vi "init.vi"(8 "error in":errorcluster, 10 "TBM module configuration in":refnum<class "TBM module configuration.lvclass">, 11 "Daqmx Module runtime in":refnum<class "Daqmx Module runtime.lvclass">) -> (0 "error out":errorcluster, 1 "data allocations":T1, 2 "execution settings":T4, 3 "Daqmx Module runtime out":refnum<class "Daqmx Module runtime.lvclass">)   [LabVIEW 2015, in "DAQmx Module Runtime.lvclass"]
doc: "Provides an interface for initializing a module at runtime. While this interface performs no operations, a child should provide an override which may open any necessary references or sessions, allocate necessary memory, and perform any final configuration validataion before providing the full configuration <b>execution data</b> to the calling process."
uses:
  Daqmx Module runtime.lvclass
  <vilib>/NI/Tag Bus Module Framework/module configuration/TBM module configuration.lvclass
  <vilib>/NI/Tag Bus Module Framework/runtime/execution settings.ctl
  <vilib>/NI/Tag Bus Module Framework/channel/data tables.ctl
  <vilib>/NI/Tag Bus/dictionary/data dictionary.lvclass
  <vilib>/NI/Tag Bus/dictionary table pair.ctl
  <vilib>/NI/Tag Bus/table/data table.ctl
  configuration/Daqmx Module configuration.lvclass
  Channel Indeces.ctl
  configuration/Daqmx Module configuration.lvclass/Daqmx Module configuration.ctl
  <vilib>/NI/Tag Bus/tag/tag descriptor.lvclass/tag descriptor.ctl
  Daqmx Module runtime.lvclass/Daqmx Module runtime.ctl
  configuration/Read Data Rate.vi
  <vilib>/NI/Tag Bus/tag/read tag name.vi
  <vilib>/NI/Tag Bus/tag/read data type.vi
  <vilib>/NI/Tag Bus/dictionary/locate tag.vi
  <vilib>/DAQmx/create/channels.llb/DAQmx Create Channel (AI-Voltage-Basic).vi
  <vilib>/DAQmx/create/channels.llb/DAQmx Create Channel (AI-Strain-Strain Gage).vi
  <vilib>/DAQmx/create/channels.llb/DAQmx Create Channel (AI-Temperature-Thermocouple).vi
  <vilib>/DAQmx/create/channels.llb/DAQmx Create Channel (AI-Current-Basic).vi
  <vilib>/DAQmx/create/channels.llb/DAQmx Create Channel (AI-Temperature-RTD).vi
  <vilib>/DAQmx/create/channels.llb/DAQmx Create Channel (AO-Current-Basic).vi
  <vilib>/DAQmx/create/channels.llb/DAQmx Create Channel (AO-Voltage-Basic).vi
  <vilib>/DAQmx/create/channels.llb/DAQmx Create Channel (DO-Digital Output).vi
  <vilib>/DAQmx/create/channels.llb/DAQmx Create Channel (CO-Pulse Generation-Frequency).vi
  <vilib>/DAQmx/create/channels.llb/DAQmx Create Channel (DI-Digital Input).vi
  <vilib>/NI/Tag Bus Module Framework/channel/TBM channel.lvclass
  <vilib>/NI/Tag Bus Module Framework/runtime/TBM module execution interface.lvclass
  <resource>/objmgr/daqmx.rc
  <vilib>/NI/Tag Bus/tag bus.lvlib
  <vilib>/NI/Tag Bus/table/data table.lvlib
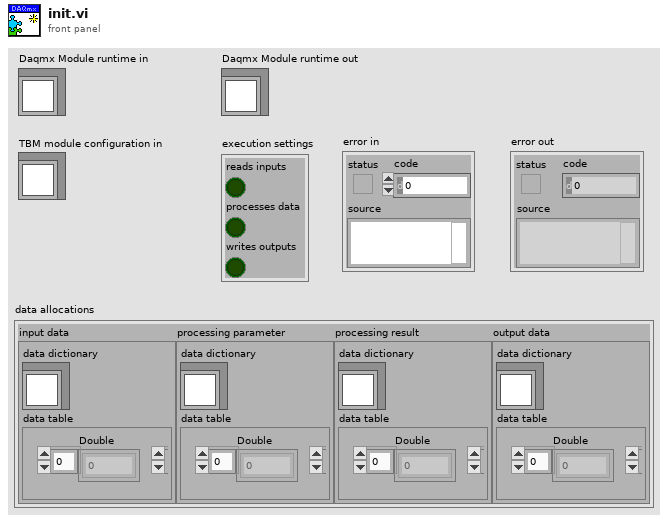
[diagram p1: front panel]
types:
  T1 = typedef "TBM channel.lvclass/data tables.ctl" = cluster{"input data":T2, "processing parameter":T2, "processing result":T2, "output data":T2}
  T2 = typedef "tag bus.lvlib/dictionary table pair.ctl" = cluster{"data dictionary":refnum<class "data dictionary.lvclass">, "data table":T3}
  T3 = typedef "tag bus.lvlib/data table.lvlib/data table.ctl" = cluster{"Double":dbl[], "Single":sgl[], "I64":i64[], "I32":i32[], "I16":i16[], "I8":i8[], "U64":u64[], "U32":u32[], "U16":u16[], "U8":u8[], "Boolean":bool[], "String":string[], "Array of Double":cluster{"DBL Array":dbl[]}[], "Array of Single":cluster{"SGL Array":sgl[]}[], "Array of I64":cluster{"I64 Array":i64[]}[], "Array of I32":cluster{"I32 Array":i32[]}[], "Array of I16":cluster{"I16 Array":i16[]}[], "Array of I8":cluster{"I8 Array":i8[]}[], "Array of U64":cluster{"U64 Array":u64[]}[], "Array of U32":cluster{"U32 Array":u32[]}[], "Array of U16":cluster{"U16 Array":u16[]}[], "Array of U8":cluster{"U8 Array":u8[]}[], "Array of Boolean":cluster{"Boolean Array":bool[]}[], "Array of String":cluster{"String Array":string[]}[]}
  T4 = typedef "TBM module execution interface.lvclass/execution settings.ctl" = cluster{"reads inputs":bool, "processes data":bool, "writes outputs":bool}
  T5 = typedef "DAQmx Module Runtime.lvclass/Channel Indeces.ctl" = cluster{"AI Index":i32[], "AO Index":i32[], "DI Index":i32[], "DO Index":i32[], "PWM Freq Index":i32[], "PWM DC Index":i32[]}
  T6 = typedef "DAQmx Module Configuration.lvclass/Line.ctl" = cluster{"Channel Array":refnum<class "TBM channel.lvclass">[], "Physical Channel":string, "Measurement Type":T7, "Parameters":T8}
  T7 = typedef "DAQmx Module Configuration.lvclass/Measurement Type.ctl" = enum16{"Digital Input", "Digital Output", "Voltage Input", "Voltage Output", "Current Input", "Current Output", "RTD", "Thermocouple", "Strain", "PWM"}
  T8 = typedef "DAQmx Module Configuration.lvclass/Parameters.ctl" = cluster{"Digital Config":cluster{"Invert Lines?":bool}, "Voltage Config":cluster{"Maximum Value (V)":dbl, "Minimum Value (V)":dbl, "in terminal configuration (V)":i32, "out terminal configuration (V)":i32}, "Current Config":cluster{"Maximum Value (A)":dbl, "Minimum Value (A)":dbl, "shunt resistor location":i32, "input terminal configuration (C)":i32, "external shunt resistor value":dbl}, "RTD Config":cluster{"Maximum Value (°C)":dbl, "Minimum Value (°C)":dbl, "resistance configuration":i32, "r0":dbl, "current excitation value":dbl, "rtd type":i32, "current excitation source":i32}, "Thermocouple Config":cluster{"Minimum Value (C)":dbl, "Maximum Value (C)":dbl, "thermocouple type":i32, "cjc source":i32, "cjc value":dbl}, "Strain Config":cluster{"Maximum Value":dbl, "Minimum Value":dbl, "bridge information":cluster{"strain configuration":i32, "lead wire resistance":dbl, "initial bridge voltage":dbl, "voltage excitation source":i32, "voltage excitation value":dbl}, "strain gage information":cluster{"gage factor":dbl, "nominal gage resistance":dbl, "poisson ratio":dbl}}, "PWM Config":cluster{"Idle State":bool}}
  T9 = typedef "DAQmx Module Runtime.lvclass/DAQ Tasks.ctl" = cluster{"AI Task":refnum<k21>, "AO Task":refnum<k21>, "DI Task":refnum<k21>, "DO Task":refnum<k21>, "PWM Task":refnum<k21>}
  T10 = cluster{"strain configuration":i32, "lead wire resistance":dbl, "initial bridge voltage":dbl, "voltage excitation source":i32, "voltage excitation value":dbl}
  T11 = cluster{"gage factor":dbl, "nominal gage resistance":dbl, "poisson ratio":dbl}
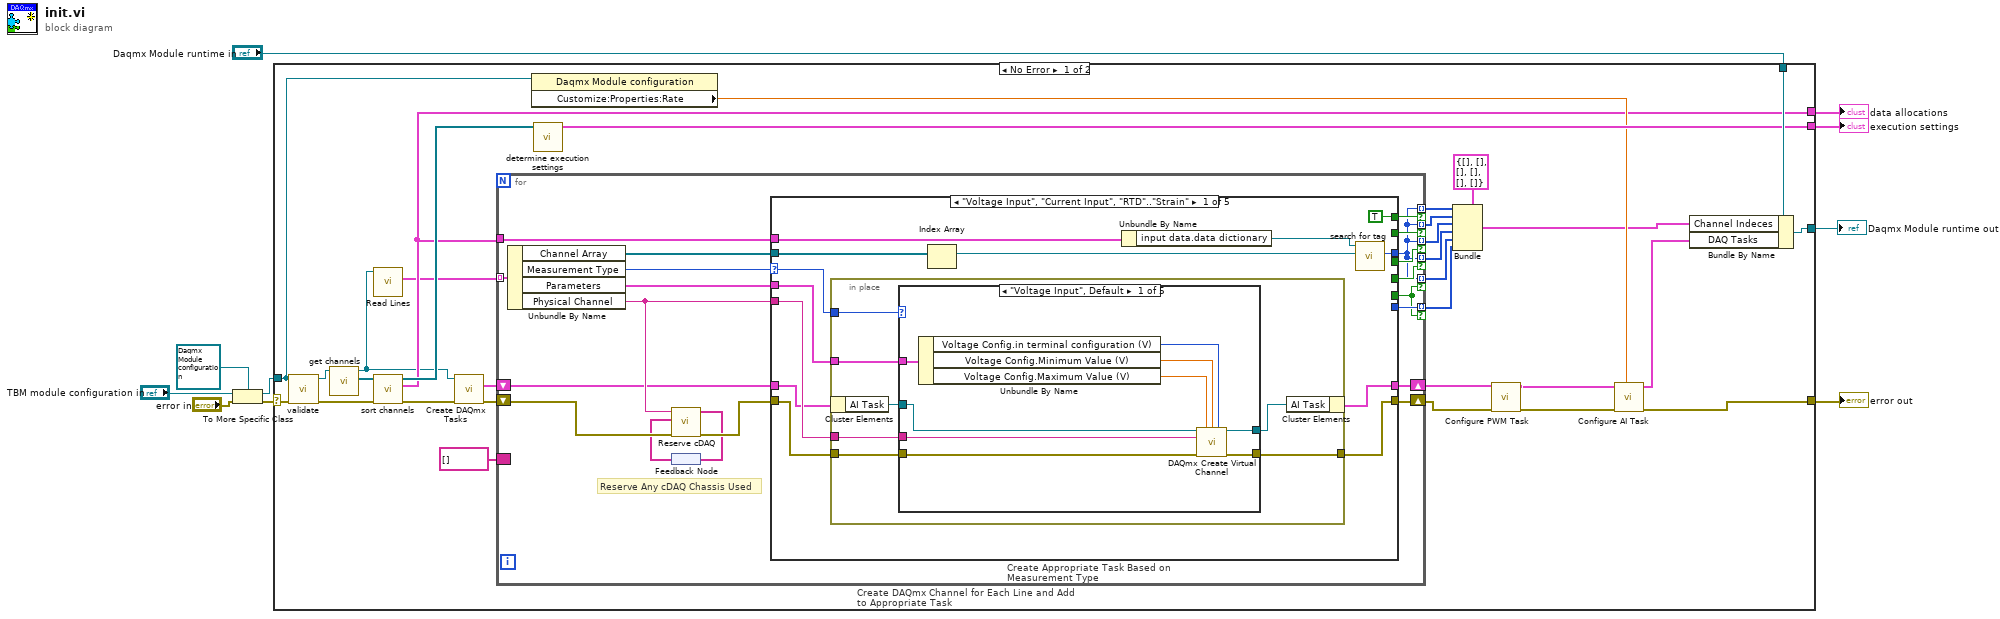
[diagram p0: block diagram]
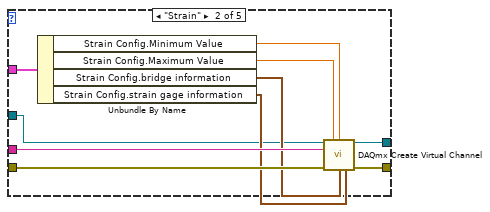
[diagram p2: hidden frame]
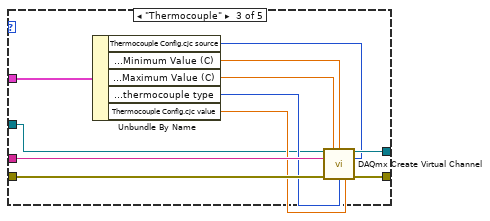
[diagram p3: hidden frame]
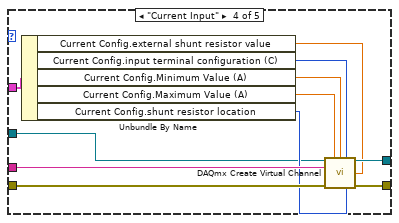
[diagram p4: hidden frame]
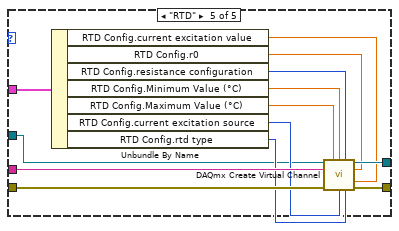
[diagram p5: hidden frame]
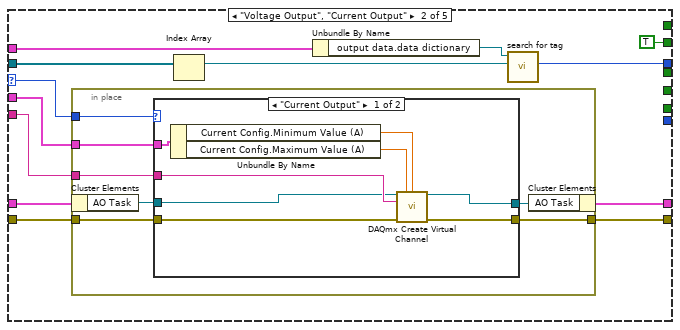
[diagram p6: hidden frame]
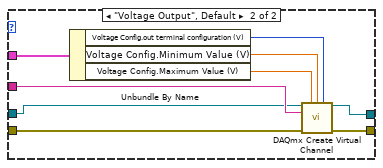
[diagram p7: hidden frame]
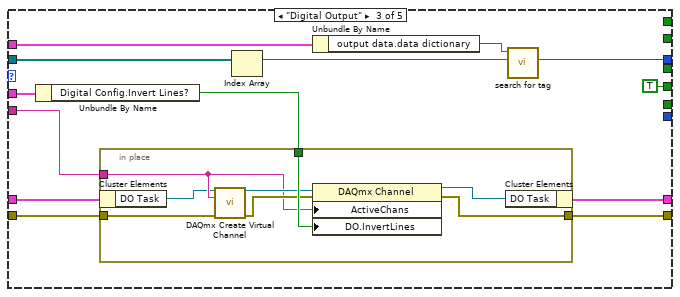
[diagram p8: hidden frame]
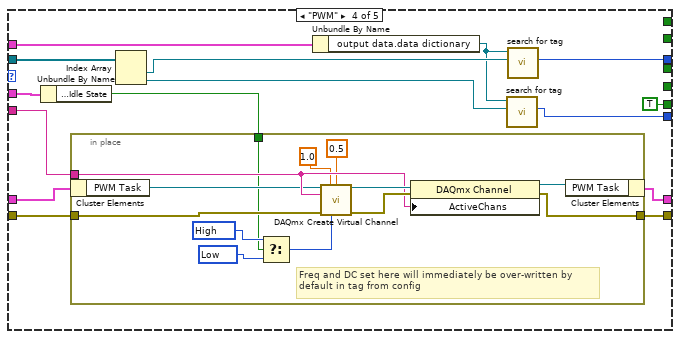
[diagram p9: hidden frame]
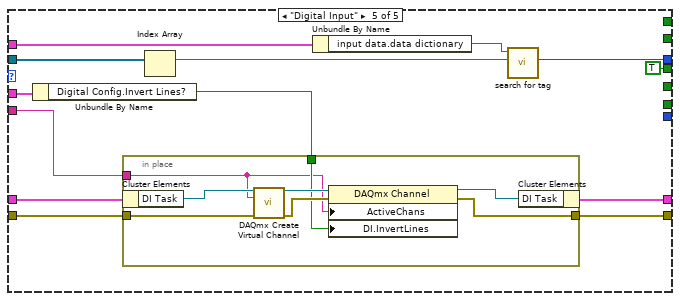
[diagram p10: hidden frame]
diagram:
  n1 = To More Specific Class(target class=refnum<class "Daqmx Module configuration.lvclass"> refnum ("Synchronous module configuration"), reference="TBM module configuration in", error in="error in") -> (specific class reference=w9:refnum<class "Daqmx Module configuration.lvclass">, error out=w10:errorcluster)
  n2 = case shown="No Error" w10 {
    selector: w10 -> [w37 w244]
    tunnel: w9 -> [w33 _]
    tunnel: "Daqmx Module runtime in" -> [w41 w243]
    tunnel: [w34 w243] -> w6
    tunnel: [w23 w244] -> w5
    tunnel: [w19 _] -> w3
    tunnel: [w40 _] -> w4
    frame No Error {
      n3 = call-dynamic "validate.vi"("error in"=w37, "Daqmx Module configuration in"=w33) -> ("error out"=w38:errorcluster, "Daqmx Module configuration out"=w36:refnum<class "Daqmx Module configuration.lvclass">)  [unwired: 8 in]
      n4 = call-dynamic "get channels.vi"("Daqmx Module configuration in"=w36) -> ("channels"=w35:refnum<class "TBM channel.lvclass">[], "Daqmx Module configuration out"=w18:refnum<class "Daqmx Module configuration.lvclass">)  [unwired: 9 in]
      n5 = call "Read Lines.vi"("Daqmx Module configuration in"=w18) -> ("Lines"=w17:T6[])  [unwired: 8 in, 2 out]
      n6 = call <vilib>:"sort channels.vi"("error in"=w38, "channels in"=w35) -> ("error out"=w32:errorcluster, "data allocations"=w19:T1, "channels out"=w39:refnum<class "TBM channel.lvclass">[])  [unwired: 7 in]
      n7 = call "Create DAQmx Tasks.vi"("Error In"=w32, "Daqmx Module configuration"=w18) -> ("Error Out"=w31:errorcluster, "DAQ Tasks"=w30:T9)  [unwired: 8 in]
      n8 = for "Create DAQmx Channel for Each Line and Add to Appropriate Task" {
        shift-right: [w49] -> w13
        shift-left: w31 -> [w51]
        tunnel: w17 -> [w61] mode=indexing
        tunnel: w19 -> [w59]
        tunnel: [w44] -> w24 mode=indexing if=w58
        tunnel: [w44] -> w25 mode=indexing if=w56
        tunnel: [w44] -> w27 mode=indexing if=w54
        tunnel: [w44] -> w26 mode=indexing if=w55
        shift-right: [w45] -> w14
        shift-left: w30 -> [w48]
        border: string[] [] -> [_]
        tunnel: [w44] -> w16 mode=indexing if=w42
        tunnel: [w43] -> w15 mode=indexing if=w42
        # "Reserve Any cDAQ Chassis Used"
        n9 = Unbundle By Name(w61) -> ("Channel Array"=w53:refnum<class "TBM channel.lvclass">[], "Measurement Type"=w60:T7, "Parameters"=w57:T8, "Physical Channel"=w52:string)
        n10 = feedback #1() -> (w46:string[])
        n11 = call "Reserve cDAQ.vi"("error in (no error)"=w51, "Array in"=w46, "Physical Channel"=w52) -> ("error out"=w50:errorcluster, "Array out"=w47:string[])  [unwired: 7 in]
        n12 = feedback-in #1(w47) -> ()
        n13 = case "Create Appropriate Task Based on Measurement Type" shown="\"Voltage Input\", \"Current Input\", \"RTD\"..\"Strain\"" w60 {
          selector: w60 -> [w68 w141 _ _ _]
          tunnel: w50 -> [w74 w148 w185 w208 w234]
          tunnel: [w66 w147 w178 w194 w228] -> w49
          tunnel: w59 -> [w73 w146 w184 w207 w233]
          tunnel: [_ _ TRUE _ _] -> w58
          tunnel: w53 -> [w72 w145 w183 w206 w232]
          tunnel: [w71 w144 w182 w205 w231] -> w44
          tunnel: w57 -> [w67 w140 w180 w201 w229]
          tunnel: [_ _ _ _ TRUE] -> w56
          tunnel: [_ TRUE _ _ _] -> w55
          tunnel: [TRUE _ _ _ _] -> w54
          tunnel: w52 -> [w69 w142 w177 w204 w227]
          tunnel: w48 -> [w65 w139 w176 w203 w225]
          tunnel: [w64 w138 w175 w202 w224] -> w45
          tunnel: [_ _ _ TRUE _] -> w42
          tunnel: [_ _ _ w195 _] -> w43
          frame "Voltage Input", "Current Input", "RTD".."Strain" {
            n14 = in-place {
              in-place-border: w74 -> [w81]
              in-place-border: w69 -> [w80]
              in-place-border: w68 -> [w79]
              in-place-border: w67 -> [w78]
              in-place-border: [w77] -> w66
              n15 = in-place-cluster #2(w65) -> ("AI Task"=w76:refnum<k21>)
              n16 = case shown="\"Voltage Input\", Default" w79 {
                tunnel: w81 -> [w90 w100 w111 w122 w135]
                tunnel: [w89 w99 w110 w121 w134] -> w77
                tunnel: [w88 w98 w109 w120 w133] -> w75
                tunnel: w80 -> [w87 w97 w108 w119 w132]
                tunnel: w78 -> [w85 w95 w106 w117 w131]
                tunnel: w76 -> [w82 w91 w101 w112 w123]
                frame "Voltage Input", Default {
                  n17 = Unbundle By Name(w85) -> ("Voltage Config.in terminal configuration (V)"=w83:i32, "Voltage Config.Minimum Value (V)"=w84:dbl, "Voltage Config.Maximum Value (V)"=w86:dbl)
                  n18 = call-poly <vilib>:"DAQmx Create Virtual Channel.vi"("task in"=w82, "maximum value"=w86, "minimum value"=w84, "input terminal configuration"=w83, "physical channels"=w87, "error in"=w90) -> ("task out"=w88:refnum<k21>, "error out"=w89:errorcluster)  [unwired: 8 in]
                }
                frame "Strain" {
                  n19 = Unbundle By Name(w95) -> ("Strain Config.Minimum Value"=w94:dbl, "Strain Config.Maximum Value"=w96:dbl, "Strain Config.bridge information"=w93:T10, "Strain Config.strain gage information"=w92:T11)
                  n20 = call-poly <vilib>:"DAQmx Create Virtual Channel.vi"("task in"=w91, "maximum value"=w96, "minimum value"=w94, "physical channels"=w97, "error in"=w100, "bridge information"=w93, "strain gage information"=w92) -> ("task out"=w98:refnum<k21>, "error out"=w99:errorcluster)  [unwired: 7 in]
                }
                frame "Thermocouple" {
                  n21 = Unbundle By Name(w106) -> ("Thermocouple Config.cjc source"=w102:i32, "Thermocouple Config.Minimum Value (C)"=w105:dbl, "Thermocouple Config.Maximum Value (C)"=w107:dbl, "Thermocouple Config.thermocouple type"=w104:i32, "Thermocouple Config.cjc value"=w103:dbl)
                  n22 = call-poly <vilib>:"DAQmx Create Virtual Channel.vi"("task in"=w101, "maximum value"=w107, "minimum value"=w105, "physical channels"=w108, "cjc source"=w102, "error in"=w111, "thermocouple type"=w104, "cjc value"=w103) -> ("task out"=w109:refnum<k21>, "error out"=w110:errorcluster)  [unwired: 6 in]
                }
                frame "Current Input" {
                  n23 = Unbundle By Name(w117) -> ("Current Config.external shunt resistor value"=w114:dbl, "Current Config.input terminal configuration (C)"=w115:i32, "Current Config.Minimum Value (A)"=w116:dbl, "Current Config.Maximum Value (A)"=w118:dbl, "Current Config.shunt resistor location"=w113:i32)
                  n24 = call-poly <vilib>:"DAQmx Create Virtual Channel.vi"("task in"=w112, "maximum value"=w118, "minimum value"=w116, "input terminal configuration"=w115, "physical channels"=w119, "external shunt resistor value"=w114, "error in"=w122, "shunt resistor location"=w113) -> ("task out"=w120:refnum<k21>, "error out"=w121:errorcluster)  [unwired: 6 in]
                }
                frame "RTD" {
                  n25 = Unbundle By Name(w131) -> ("RTD Config.current excitation value"=w126:dbl, "RTD Config.r0"=w125:dbl, "RTD Config.resistance configuration"=w128:i32, "RTD Config.Minimum Value (°C)"=w129:dbl, "RTD Config.Maximum Value (°C)"=w130:dbl, "RTD Config.current excitation source"=w127:i32, "RTD Config.rtd type"=w124:i32)
                  n26 = call-poly <vilib>:"DAQmx Create Virtual Channel.vi"("task in"=w123, "maximum value"=w130, "minimum value"=w129, "resistance configuration"=w128, "physical channels"=w132, "r0"=w125, "current excitation value"=w126, "error in"=w135, "current excitation source"=w127, "rtd type"=w124) -> ("task out"=w133:refnum<k21>, "error out"=w134:errorcluster)  [unwired: 4 in]
                }
              }
              n27 = in-place-cluster #2("AI Task"=w75) -> (w64:T9)
            }
            n28 = Index Array(array=w72) -> (element=w62:refnum<class "TBM channel.lvclass">)  [unwired: 1 in]
            n29 = Unbundle By Name(w73) -> ("input data.data dictionary"=w70:refnum<class "data dictionary.lvclass">)
            n30 = call <vilib>:"search for tag.vi"("system tag"=w62, "data dictionary in"=w70) -> ("index"=w71:i32)  [unwired: 7 in, 2 out]
          }
          frame "Voltage Output", "Current Output" {
            n31 = in-place {
              in-place-border: w148 -> [w155]
              in-place-border: [w154] -> w147
              in-place-border: w142 -> [w153]
              in-place-border: w141 -> [w152]
              in-place-border: w140 -> [w151]
              n32 = in-place-cluster #3(w139) -> ("AO Task"=w149:refnum<k21>)
              n33 = case shown="\"Current Output\"" w152 {
                tunnel: w155 -> [w163 w172]
                tunnel: [w162 w171] -> w150
                tunnel: [w161 w170] -> w154
                tunnel: w153 -> [w160 w169]
                tunnel: w151 -> [w159 w168]
                tunnel: w149 -> [w156 w164]
                frame "Current Output" {
                  n34 = Unbundle By Name(w159) -> ("Current Config.Minimum Value (A)"=w157:dbl, "Current Config.Maximum Value (A)"=w158:dbl)
                  n35 = call-poly <vilib>:"DAQmx Create Virtual Channel.vi"("task in"=w156, "maximum value"=w158, "minimum value"=w157, "physical channels"=w160, "error in"=w163) -> ("task out"=w162:refnum<k21>, "error out"=w161:errorcluster)  [unwired: 9 in]
                }
                frame "Voltage Output", Default {
                  n36 = Unbundle By Name(w168) -> ("Voltage Config.out terminal configuration (V)"=w165:i32, "Voltage Config.Minimum Value (V)"=w166:dbl, "Voltage Config.Maximum Value (V)"=w167:dbl)
                  n37 = call-poly <vilib>:"DAQmx Create Virtual Channel.vi"("task in"=w164, "maximum value"=w167, "minimum value"=w166, "output terminal configuration"=w165, "physical channels"=w169, "error in"=w172) -> ("task out"=w171:refnum<k21>, "error out"=w170:errorcluster)  [unwired: 8 in]
                }
              }
              n38 = in-place-cluster #3("AO Task"=w150) -> (w138:T9)
            }
            n39 = Index Array(array=w145) -> (element=w136:refnum<class "TBM channel.lvclass">)  [unwired: 1 in]
            n40 = Unbundle By Name(w146) -> ("output data.data dictionary"=w143:refnum<class "data dictionary.lvclass">)
            n41 = call <vilib>:"search for tag.vi"("system tag"=w136, "data dictionary in"=w143) -> ("index"=w144:i32)  [unwired: 7 in, 2 out]
          }
          frame "Digital Output" {
            n42 = Unbundle By Name(w180) -> ("Digital Config.Invert Lines?"=w179:bool)
            n43 = in-place {
              in-place-border: w185 -> [w193]
              in-place-border: w179 -> [w192]
              in-place-border: [w189] -> w178
              in-place-border: w177 -> [w188]
              n44 = in-place-cluster #4(w176) -> ("DO Task"=w187:refnum<k21>)
              n45 = call-poly <vilib>:"DAQmx Create Virtual Channel.vi"("task in"=w187, "lines"=w188, "error in"=w193) -> ("task out"=w190:refnum<k21>, "error out"=w191:errorcluster)  [unwired: 11 in]
              n46 = property class="DAQmx Channel"(reference=w190, error in=w191, "ActiveChans"=w188, "DO.InvertLines"=w192) -> (reference out=w186:refnum<k21>, error out=w189:errorcluster)
              n47 = in-place-cluster #4("DO Task"=w186) -> (w175:T9)
            }
            n48 = Index Array(array=w183) -> (element=w173:refnum<class "TBM channel.lvclass">)  [unwired: 1 in]
            n49 = Unbundle By Name(w184) -> ("output data.data dictionary"=w181:refnum<class "data dictionary.lvclass">)
            n50 = call <vilib>:"search for tag.vi"("system tag"=w173, "data dictionary in"=w181) -> ("index"=w182:i32)  [unwired: 7 in, 2 out]
          }
          frame "PWM" {
            n51 = Unbundle By Name(w201) -> ("PWM Config.Idle State"=w200:bool)
            n52 = in-place {
              in-place-border: w208 -> [w221]
              in-place-border: w204 -> [w218]
              in-place-border: w200 -> [w214]
              in-place-border: [w212] -> w194
              w213 = 10214 items=["High"=10192, "Low"=10214] ("idle state")
              w216 = 10192 items=["High"=10192, "Low"=10214] ("idle state")
              # "Freq and DC set here will immediately be over-written by\ndefault in tag from config"
              n53 = in-place-cluster #5(w203) -> ("PWM Task"=w217:refnum<k21>)
              n54 = Select(t=w216, s=w214, f=w213) -> (s? t:f=w215:i32)
              n55 = call-poly <vilib>:"DAQmx Create Virtual Channel.vi"("task in"=w217, "frequency"=1.0, "duty cycle"=0.5, "counter"=w218, "error in"=w221, "idle state"=w215) -> ("task out"=w219:refnum<k21>, "error out"=w220:errorcluster)  [unwired: 8 in]
              n56 = property class="DAQmx Channel"(reference=w219, error in=w220, "ActiveChans"=w218) -> (reference out=w211:refnum<k21>, error out=w212:errorcluster)
              n57 = in-place-cluster #5("PWM Task"=w211) -> (w202:T9)
            }
            n58 = Index Array(array=w206) -> (element #1=w198:refnum<class "TBM channel.lvclass">, element #2=w196:refnum<class "TBM channel.lvclass">)  [unwired: 2 in]
            n59 = Unbundle By Name(w207) -> ("output data.data dictionary"=w197:refnum<class "data dictionary.lvclass">)
            n60 = call <vilib>:"search for tag.vi"("system tag"=w196, "data dictionary in"=w197) -> ("index"=w195:i32)  [unwired: 7 in, 2 out]
            n61 = call <vilib>:"search for tag.vi"("system tag"=w198, "data dictionary in"=w197) -> ("index"=w205:i32)  [unwired: 7 in, 2 out]
          }
          frame "Digital Input" {
            n62 = Unbundle By Name(w229) -> ("Digital Config.Invert Lines?"=w226:bool)
            n63 = in-place {
              in-place-border: w234 -> [w242]
              in-place-border: [w239] -> w228
              in-place-border: w227 -> [w235]
              in-place-border: w226 -> [w238]
              n64 = in-place-cluster #6(w225) -> ("DI Task"=w237:refnum<k21>)
              n65 = call-poly <vilib>:"DAQmx Create Virtual Channel.vi"("task in"=w237, "lines"=w235, "error in"=w242) -> ("task out"=w241:refnum<k21>, "error out"=w240:errorcluster)  [unwired: 11 in]
              n66 = property class="DAQmx Channel"(reference=w241, error in=w240, "ActiveChans"=w235, "DI.InvertLines"=w238) -> (reference out=w236:refnum<k21>, error out=w239:errorcluster)
              n67 = in-place-cluster #6("DI Task"=w236) -> (w224:T9)
            }
            n68 = Index Array(array=w232) -> (element=w222:refnum<class "TBM channel.lvclass">)  [unwired: 1 in]
            n69 = Unbundle By Name(w233) -> ("input data.data dictionary"=w230:refnum<class "data dictionary.lvclass">)
            n70 = call <vilib>:"search for tag.vi"("system tag"=w222, "data dictionary in"=w230) -> ("index"=w231:i32)  [unwired: 7 in, 2 out]
          }
        }
      }
      n71 = property class="Daqmx Module configuration"(reference=w33) -> ("Customize:Properties:Rate"=w22:dbl)  [unwired: 1 in, 2 out]
      n72 = call <vilib>:"determine execution settings.vi"("channels"=w39) -> ("execution settings"=w40:T4)  [unwired: 10 in]
      n73 = Bundle(cluster=T5 {"AI Index"=[], "AO Index"=[], "DI Index"=[], "DO Index"=[], "PWM Freq Index"=[], "PWM DC Index"=[]} ("Channel Indeces"), "AI Index"=w27, "AO Index"=w26, "DI Index"=w25, "DO Index"=w24, "PWM Freq Index"=w16, "PWM DC Index"=w15) -> (w21:T5)
      n74 = call "Configure PWM Task.vi"("error in (no error)"=w13, "DAQ Tasks"=w14) -> ("error out"=w12:errorcluster, "DAQ Tasks Out"=w11:T9)  [unwired: 8 in]
      n75 = call "Configure AI Task.vi"("Sampling Rate"=w22, "error in (no error)"=w12, "DAQ Tasks in"=w11) -> ("error out"=w23:errorcluster, "DAQ Tasks out"=w20:T9)  [unwired: 7 in]
      n76 = Bundle By Name(cluster=w41, "Channel Indeces"=w21, "DAQ Tasks"=w20) -> (w34:refnum<class "Daqmx Module runtime.lvclass">)
    }
    frame Error {
    }
  }
  "error out" <- w5
  "Daqmx Module runtime out" <- w6
  "execution settings" <- w4
  "data allocations" <- w3
